vi "Notification LED.vi"(8 "error in":errorcluster) -> (0 "error out":errorcluster, 2 "Result":string, 3 "RESULT":bool)   [LabVIEW 2021]
uses:
  DUT/DUT_Cmd.ctl
panel:
  in  "PCB Serial No":string
  out "Command Response":string
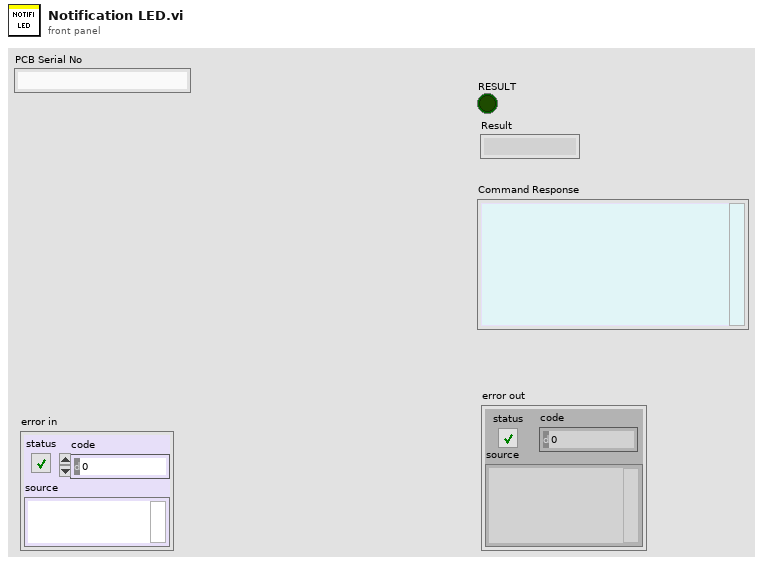
[diagram p1: front panel]
types:
  T1 = typedef "DUT_Cmd.ctl" = enum16{"Unlock serial", "Stop console logs", "Release emergency at start", "Read firmware", "WiFi credentials", "WiFi connected", "WiFi SSID", "Board revision", "ADC_NTC_TEMP", "ADC_TYPE2_RCD_CURRENT", "PCBA serial write", "PCBA serial readback", "Start energy meter", "Energy meter Vac", "Energy meter Iac", "Energy meter PF", "Energy meter energy", "Provision", "Set gateway identity", "CP checklist", "Earth detect", "D+M sense unplugged", "D+M sense plugged", "Output relay weld", "Start diagnostics", "Relay 1 on", "Relay 2 on", "Emergency pressed", "Release emergency", "Emergency released", "Unlock serial for 5 A", "Board current (5 A)", "Unlock serial for 15 A", "Board current (15 A)", "Unlock serial for 0 A", "NFC tag", "Start diagnostics again", "Relay 2 off", "Relay 1 off", "End diagnostics", "Load current (5 A) [No USB station]", "Load current (15 A) [No USB station]", "Load current (0 A) [No USB station]", "NFC tag [No USB station]", "Battery Voltage", "FW Power reset", "Notification LED", "O/P Relay weld Detection", "Earth Detection", "12V ", "5V", "3.3V"}
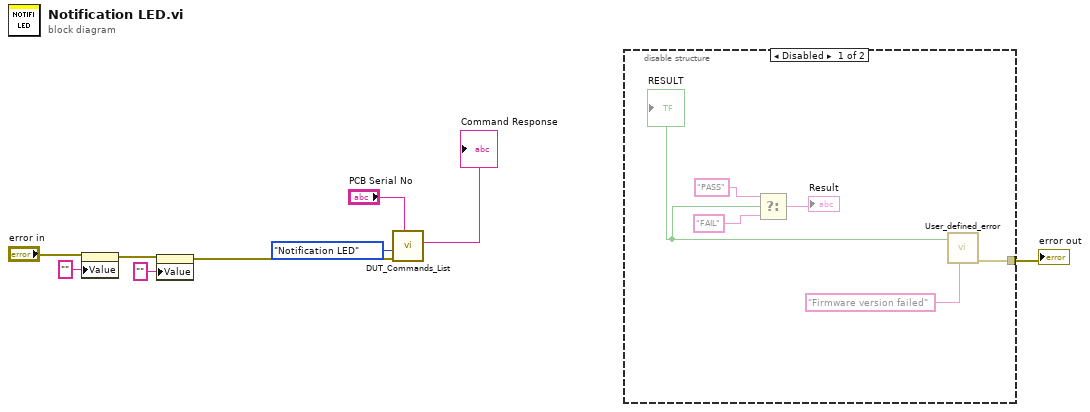
[diagram p0: block diagram]
diagram:
  n1 = property on="PCB Serial No" class="Str"(error in="error in", "Value"="" ("PCB Serial No")) -> (error out=w2:errorcluster)  [unwired: 1 in, 1 out]
  n2 = property on="Command Response" class="Str"(error in=w2, "Value"="" ("Command Response")) -> (error out=w7:errorcluster)  [unwired: 1 in, 1 out]
  n3 = call "DUT_Commands_List.vi"("PCB Serial No"="PCB Serial No", "error in"=w7, "DUT Cmd"=DUT_Cmd."Notification LED") -> ("Command Response"=→"Command Response":string)  [unwired: 6 in, 2 out]
  n4 = disable-structure shown="Disabled" {
    disable-tunnel: [w14 _] -> w9
    frame Disabled {
      n5 = call "User_defined_error.vi"("Error Msg"="Firmware version failed" ("source")) -> ("error Out"=w14:errorcluster, "Result"=w13:bool)  [unwired: 9 in]
      "RESULT" <- w13
      n6 = Select(t="PASS", s=w13, f="FAIL") -> (s? t:f=→"Result":string)
    }
    frame Enabled {
    }
  }
  "error out" <- w9
